vi "RemoteVI Check Frame Encode.vi"() -> (4 "labels":string[](array[string]), 6 "expected":string[](array[string]), 8 "actual":string[](array[string]), 10 "failures":i32)   [LabVIEW 2020]
doc: "Test support, generated by tests/caraya/build.py from tests/vectors/frame.json - do not edit. Calls RemoteVI Frame Encode.vi once per vector: the png fields are hex in the vector and decoded to bytes before the call; the message is compared as lowercase hex. Outputs, one element per vector: labels (the vector's name), expected (rendered from the vector), actual (the VI's result rendered the same way), and failures, the number of vectors whose expected and actual differ."
uses:
  source/RemoteVI.lvlib
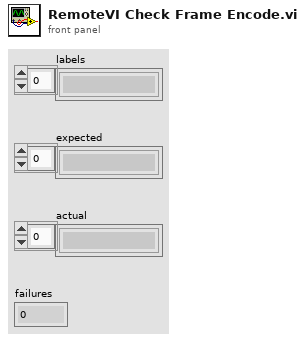
[diagram p1: front panel]
types:
  T1 = cluster{"name":string, "seq":u32, "width":u16, "height":u16, "rects":cluster{"x":i16, "y":i16, "png":string}[], "message":string}[]
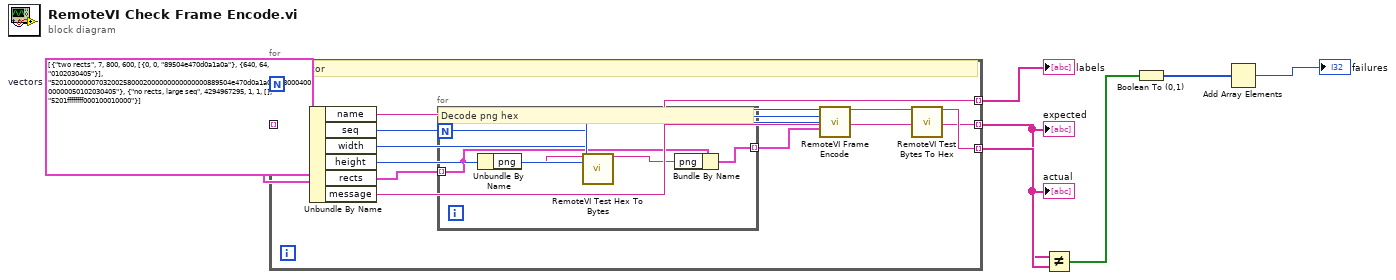
[diagram p0: block diagram]
diagram:
  w1 = T1 [{"name"="two rects", "seq"=7, "width"=800, "height"=600, "rects"=[{"x"=0, "y"=0, "png"="89504e470d0a1a0a"}, {"x"=640, "y"=64, "png"="0102030405"}], "message"="520100000007032002580002000000000000000889504e470d0a1a0a02800040000000050102030405"}, {"name"="no rects, large seq", "seq"=4294967295, "width"=1, "height"=1, "rects"=[], "message"="5201ffffffff000100010000"}]  # vectors
  n1 = for {
    tunnel: w1 -> [w8] mode=indexing
    tunnel: [w9] -> w2 mode=indexing
    tunnel: [w14] -> w3 mode=indexing
    tunnel: [w17] -> w4 mode=indexing
    # "One vector"
    n2 = Unbundle By Name(w8) -> ("name"=w9:string, "seq"=w10:u32, "width"=w11:u16, "height"=w12:u16, "rects"=w13:cluster{"x":i16, "y":i16, "png":string}[], "message"=w14:string)
    n3 = for {
      tunnel: w13 -> [w18] mode=indexing
      tunnel: [w21] -> w15 mode=indexing
      # "Decode png hex"
      n4 = Unbundle By Name(w18) -> ("png"=w19:string)
      n5 = call "RemoteVI Test Hex To Bytes.vi"("hex"=w19) -> ("bytes"=w20:string)  [unwired: 14 in]
      n6 = Bundle By Name(cluster=w18, "png"=w20) -> (w21:cluster{"x":i16, "y":i16, "png":string})
    }
    n7 = call "RemoteVI Frame Encode.vi"("seq"=w10, "width"=w11, "height"=w12, "rects"=w15) -> ("message"=w16:string)  [unwired: 11 in]
    n8 = call "RemoteVI Test Bytes To Hex.vi"("bytes"=w16) -> ("hex"=w17:string)  [unwired: 14 in]
  }
  "labels" <- w2
  "expected" <- w3
  "actual" <- w4
  n9 = Not Equal?(x=w3, y=w4) -> (x != y?=w5:bool[])
  n10 = Boolean To (0,1)(Boolean=w5) -> (0, 1=w6:i16[])
  n11 = Add Array Elements(numeric array=w6) -> (sum=→"failures":i16)
